vi "onCreateDebugTerminal.vi"(8 "error in (no error)":errorcluster, 11 "DebuggingTerminal in":refnum<class "DebuggingTerminal.lvclass">) -> (0 "error out":errorcluster, 3 "DebuggingTerminal out":refnum<class "DebuggingTerminal.lvclass">)   [LabVIEW 2013, in "MQTT Base.lvlib" / "DebuggingTerminal.lvclass"]
uses:
  DebuggingTerminal.lvclass
  Stream Data -- cluster.ctl
  DebuggingTerminal.lvclass/DebuggingTerminal.ctl
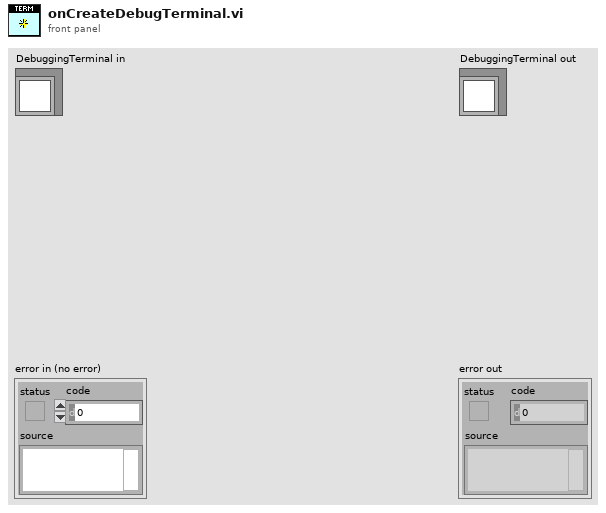
[diagram p1: front panel]
types:
  T1 = typedef "MQTT Base.lvlib/DebuggingTerminal.lvclass/Stream Data -- cluster.ctl" = cluster{"Session ID":i32, "Bytes":u8[]}
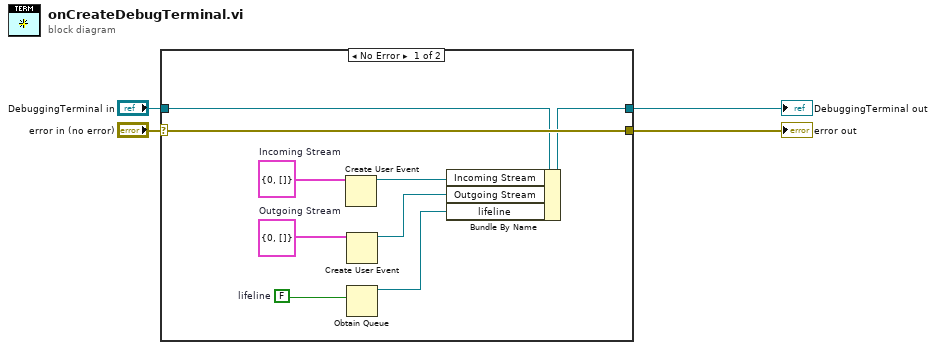
[diagram p0: block diagram]
diagram:
  n1 = case shown="No Error" "error in (no error)" {
    selector: "error in (no error)" -> [w13 w15]
    tunnel: [w13 w15] -> w3
    tunnel: [w9 w14] -> w1
    tunnel: "DebuggingTerminal in" -> [w12 w14]
    frame No Error {
      w5 = T1 {"Session ID"=0, "Bytes"=[]}  # Outgoing Stream
      w6 = T1 {"Session ID"=0, "Bytes"=[]}  # Incoming Stream
      w8 = FALSE  # lifeline
      n2 = Create User Event(user event datatype=w6) -> (user event=w11:refnum<user-event>)  [unwired: 1 in, 1 out]
      n3 = Create User Event(user event datatype=w5) -> (user event=w10:refnum<user-event>)  [unwired: 1 in, 1 out]
      n4 = Obtain Queue(element data type=w8) -> (queue out=w7:refnum<queue>)  [unwired: 4 in, 2 out]
      n5 = Bundle By Name(cluster=w12, "Incoming Stream"=w11, "Outgoing Stream"=w10, "lifeline"=w7) -> (w9:refnum<class "DebuggingTerminal.lvclass">)
    }
    frame Error {
    }
  }
  "error out" <- w3
  "DebuggingTerminal out" <- w1
